vi "Enumerate Chassis.vi"(6 "Map":map{string, T1}(c390), 8 "error in (no error)":errorcluster, 10 "Chassis Info":T1, 11 "System Element":refnum<class "Config Element.lvclass">) -> (0 "error out":errorcluster, 2 "Chassis Element":refnum<class "Config Element.lvclass">)   [LabVIEW 2020, in "Volatus.lvlib" / "Hardware Info Module.lvclass"]
uses:
  Hardware Info Module.lvclass
  lv-cdm/CDM-Config/Config Element/Config Element.lvclass
  Hardware Info Module.lvclass/Hardware Info Module.ctl
  9117e1a3-44df-4d41-bfd4-07b4189bcc33.vi
  HW Info.ctl
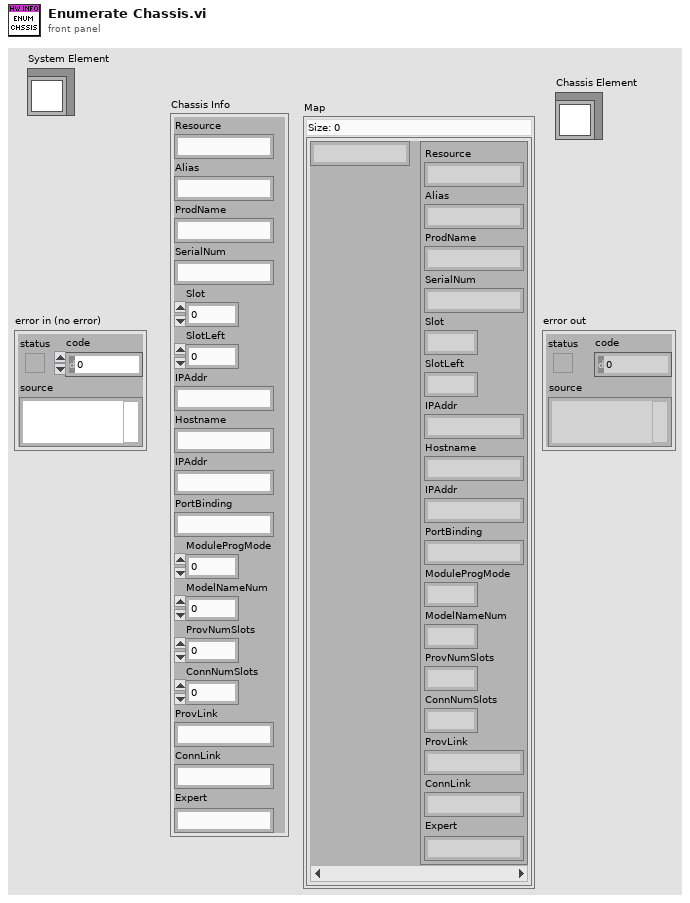
[diagram p1: front panel]
types:
  T1 = typedef "Volatus.lvlib/Hardware Info Module.lvclass/HW Info.ctl" = cluster{"Resource":string, "Alias":string, "ProdName":string, "SerialNum":string, "Slot":i32, "SlotLeft":u32, "IPAddr":string, "Hostname":string, "IPAddr":string, "PortBinding":string, "ModuleProgMode":u32, "ModelNameNum":u32, "ProvNumSlots":i32, "ConnNumSlots":i32, "ProvLink":string, "ConnLink":string, "Expert":string}
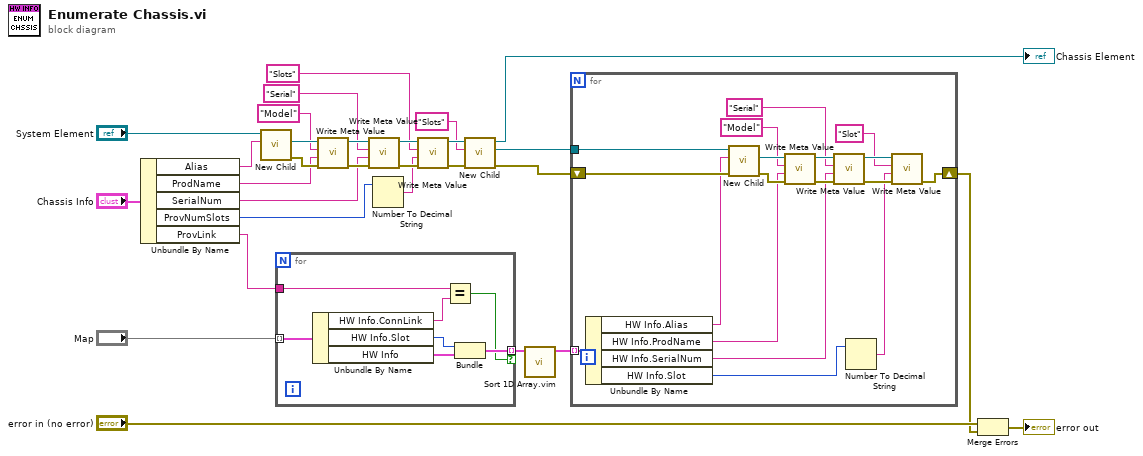
[diagram p0: block diagram]
diagram:
  n1 = Unbundle By Name("Chassis Info") -> ("Alias"=w22:string, "ProdName"=w19:string, "SerialNum"=w14:string, "ProvNumSlots"=w10:i32, "ProvLink"=w25:string)
  n2 = call "New Child.vi"("Child Name"=w22, "Config Element in"="System Element") -> ("error out"=w28:errorcluster, "New Child"=w21:refnum<class "Config Element.lvclass">)  [unwired: 7 in, 1 out]
  n3 = for {
    tunnel: w25 -> [w33]
    tunnel: "Map" -> [w35] mode=indexing
    tunnel: [w32] -> w18 mode=indexing if=w31
    n4 = Unbundle By Name(w35) -> ("HW Info.ConnLink"=w34:string, "HW Info.Slot"=w36:i32, "HW Info"=w30:T1)
    n5 = Equal?(x=w33, y=w34) -> (x = y?=w31:bool)
    n6 = Bundle("Slot"=w36, "HW Info"=w30) -> (w32:cluster{"Slot":i32, "HW Info":T1})  [unwired: 1 in]
  }
  n7 = call "Write Meta Value.vi"("error in (no error)"=w28, "Meta Value"=w19, "Meta Name"="Model", "Config Element in"=w21) -> ("error out"=w29:errorcluster, "Config Element out"=w16:refnum<class "Config Element.lvclass">)  [unwired: 6 in]
  n8 = call "Write Meta Value.vi"("error in (no error)"=w29, "Meta Value"=w14, "Meta Name"="Serial", "Config Element in"=w16) -> ("error out"=w12:errorcluster, "Config Element out"=w13:refnum<class "Config Element.lvclass">)  [unwired: 6 in]
  n9 = Number To Decimal String(number=w10) -> (decimal integer string=w9:string)  [unwired: 1 in]
  n10 = call "Write Meta Value.vi"("error in (no error)"=w12, "Meta Value"=w9, "Meta Name"="Slots", "Config Element in"=w13) -> ("error out"=w6:errorcluster, "Config Element out"=w8:refnum<class "Config Element.lvclass">)  [unwired: 6 in]
  n11 = call "New Child.vi"("error in (no error)"=w6, "Child Name"="Slots" ("Meta Name"), "Config Element in"=w8) -> ("error out"=w4:errorcluster, "New Child"=w5:refnum<class "Config Element.lvclass">, "Config Element out"=→"Chassis Element":refnum<class "Config Element.lvclass">)  [unwired: 6 in]
  n12 = call "Sort 1D Array.vim"("unsorted array"=w18) -> ("sorted array"=w17:cluster{"Slot":i32, "HW Info":T1}[])  [unwired: 10 in]
  n13 = for {
    tunnel: w17 -> [w53] mode=indexing
    tunnel: w5 -> [w52]
    shift-right: [w37] -> w2
    shift-left: w4 -> [w54]
    n14 = Unbundle By Name(w53) -> ("HW Info.Alias"=w51:string, "HW Info.ProdName"=w47:string, "HW Info.SerialNum"=w43:string, "HW Info.Slot"=w42:i32)
    n15 = call "New Child.vi"("error in (no error)"=w54, "Child Name"=w51, "Config Element in"=w52) -> ("error out"=w49:errorcluster, "New Child"=w50:refnum<class "Config Element.lvclass">)  [unwired: 6 in, 1 out]
    n16 = call "Write Meta Value.vi"("error in (no error)"=w49, "Meta Value"=w47, "Meta Name"="Model", "Config Element in"=w50) -> ("error out"=w45:errorcluster, "Config Element out"=w46:refnum<class "Config Element.lvclass">)  [unwired: 6 in]
    n17 = call "Write Meta Value.vi"("error in (no error)"=w45, "Meta Value"=w43, "Meta Name"="Serial", "Config Element in"=w46) -> ("error out"=w40:errorcluster, "Config Element out"=w41:refnum<class "Config Element.lvclass">)  [unwired: 6 in]
    n18 = Number To Decimal String(number=w42) -> (decimal integer string=w38:string)  [unwired: 1 in]
    n19 = call "Write Meta Value.vi"("error in (no error)"=w40, "Meta Value"=w38, "Meta Name"="Slot", "Config Element in"=w41) -> ("error out"=w37:errorcluster)  [unwired: 6 in, 1 out]
  }
  n20 = Merge Errors("error in (no error)", w2) -> (→"error out":errorcluster)
